vi "NI32LV2612f2ASD2_Untitled 3.vi"() -> ()   [LabVIEW 2026]
panel:
  in  "Boolean 5":bool
  in  "Boolean 4":bool
  in  "Boolean 3":bool
  out "Boolean 2":bool
  out "Boolean":bool
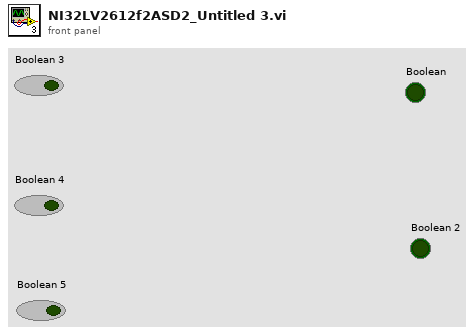
[diagram p1: front panel]
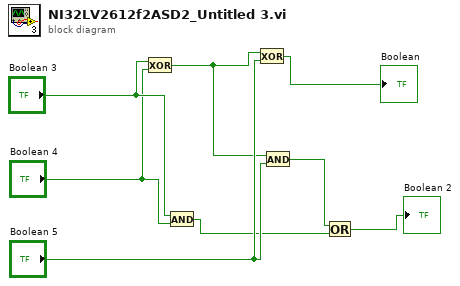
[diagram p0: block diagram]
diagram:
  n1 = Exclusive Or(1:"Boolean 4", 2:"Boolean 3") -> (0:w4:bool)
  n2 = And(x="Boolean 3", y="Boolean 4") -> (x .and. y?=w2:bool)
  n3 = Exclusive Or(1:"Boolean 5", 2:w4) -> (0:→"Boolean":bool)
  n4 = And(x=w4, y="Boolean 5") -> (x .and. y?=w3:bool)
  n5 = Or(x=w3, y=w2) -> (x .or. y?=→"Boolean 2":bool)
